vi "Check Help.vi"(8 "error in (no error)":errorcluster, 11 "LV Argument Parser in":refnum<class "LV Argument Parser.lvclass">) -> (0 "error out":errorcluster, 2 "Output":string, 3 "LV Argument Parser out":refnum<class "LV Argument Parser.lvclass">)   [LabVIEW 2020, in "LV ArgParse.lvlib" / "LV Argument Parser.lvclass"]
uses:
  LV Argument Parser.lvclass
  LV Argument Parser.lvclass/LV Argument Parser.ctl
  Get Bool.vi
  LV ArgParse.lvlib
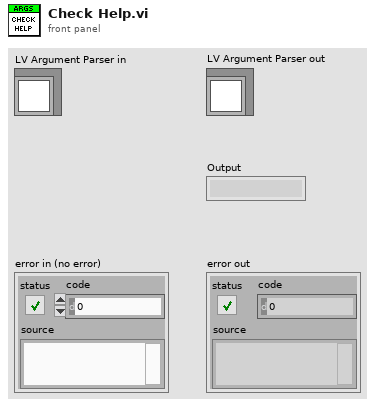
[diagram p1: front panel]
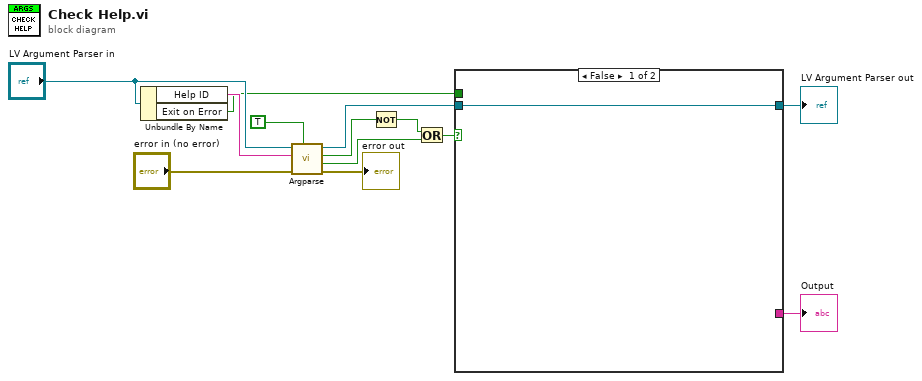
[diagram p0: block diagram]
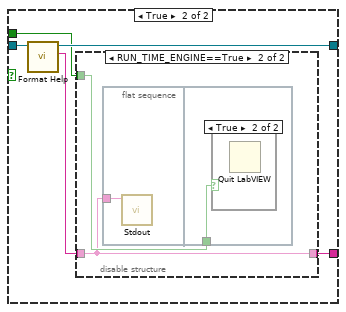
[diagram p2: hidden frame]
diagram:
  n1 = Unbundle By Name("LV Argument Parser in") -> ("Help ID"=w12:string, "Exit on Error"=w3:bool)
  n2 = call-poly "Argparse.vi"("Optional"=TRUE, "error in (no error)"="error in (no error)", "Name"=w12, "LV Argument Parser in"="LV Argument Parser in") -> ("error out"=→"error out":errorcluster, "Value"=w9:bool, "key not found?"=w5:bool, "LV Argument Parser out"=w8:refnum<class "LV Argument Parser.lvclass">)  [unwired: 4 in]
  n3 = Not(x=w5) -> (.not. x?=w4:bool)
  n4 = Or(x=w4, y=w9) -> (x .or. y?=w6:bool)
  n5 = case shown="False" w6 {
    tunnel: w8 -> [w14 w18]
    tunnel: [_ w17] -> w13
    tunnel: [w14 w16] -> w7
    tunnel: w3 -> [_ w15]
    frame False {
    }
    frame True {
      n6 = call "Format Help.vi"("LV Argument Parser in"=w18) -> ("String"=w19:string, "LV Argument Parser out"=w16:refnum<class "LV Argument Parser.lvclass">)  [unwired: 8 in, 1 out]
      n7 = disable-structure shown="RUN_TIME_ENGINE==True" {
        disable-tunnel: w19 -> [w20 w21]
        disable-tunnel: [w20 w21] -> w17
        disable-tunnel: w15 -> [_ w22]
        frame condition #0 (active) {
        }
        frame condition #1 {
          n8 = flat-sequence {
            tunnel: w21 -> [w23]
            tunnel: w22 -> [w24]
            frame #0 {
              n9 = call "Stdout.vi"("text"=w23) -> ()  [unwired: 10 in, 1 out]
            }
            frame #1 {
              n10 = case shown="True" w24 {
                frame False {
                }
                frame True {
                  n11 = Quit LabVIEW() -> ()  [unwired: 1 in]
                }
              }
            }
          }
        }
      }
    }
  }
  "LV Argument Parser out" <- w7
  "Output" <- w13
